vi "libssh2_channel_request_pty_ex.vi"(4 "height_px":i32, 5 "height":i32=24, 6 "width_px":i32, 7 "width":i32=80, 8 "error in (no error)":errorcluster, 9 "modes":string, 10 "term":string, 11 "channel":T1) -> (0 "error out":errorcluster)   [LabVIEW 2017, in "libssh2.lvlib"]
doc: "Request a pseudo-terminal on a channel."
uses:
  libssh2.lvlib
  Channel Refnum.ctl
  Acquire Session.vi
  Release Session.vi
  Not A Channel.vi
  <vilib>/Utility/error.llb/Error Cluster From Error Code.vi
  Global Settings.vi
  Read Channel Refnum.vi
  Read Session Refnum.vi
  <vilib>/Utility/semaphor.llb/Acquire Semaphore.vi
  <vilib>/Utility/semaphor.llb/Release Semaphore.vi
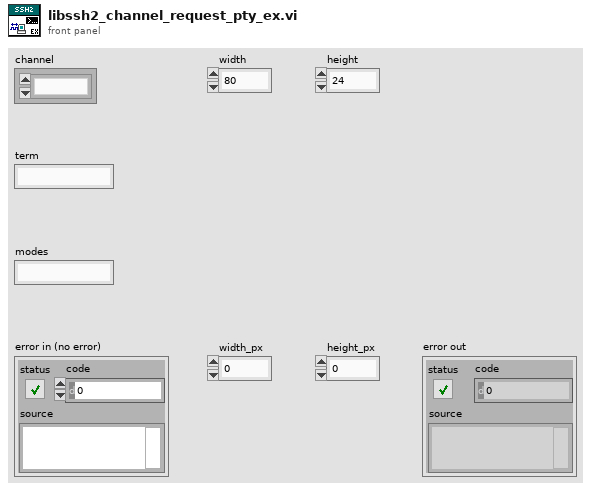
[diagram p1: front panel]
types:
  T1 = typedef "libssh2.lvlib/Channel Refnum.ctl" = refnum<k1>
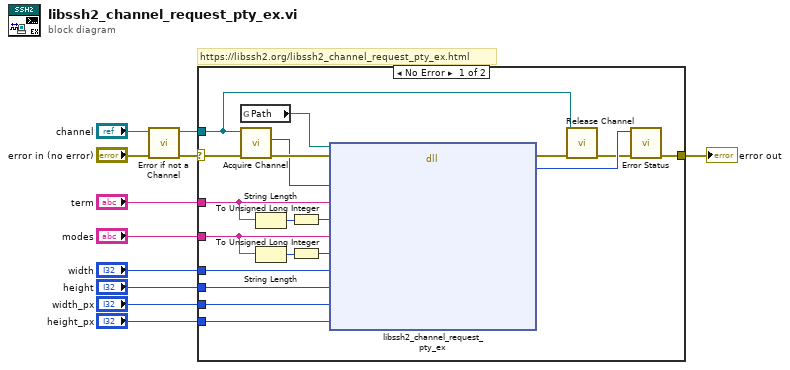
[diagram p0: block diagram]
diagram:
  # "https://libssh2.org/libssh2_channel_request_pty_ex.html"
  n1 = call "Error if not a Channel.vi"("error in (no error)"="error in (no error)", "channel"="channel") -> ("error out"=w9:errorcluster, "channel out"=w7:T1)  [unwired: 8 in]
  n2 = case shown="No Error" w9 {
    selector: w9 -> [w30 w31]
    tunnel: [w29 w31] -> w11
    tunnel: w7 -> [w12 _]
    tunnel: "term" -> [w14 _]
    tunnel: "modes" -> [w18 _]
    tunnel: "width" -> [w23 _]
    tunnel: "height" -> [w22 _]
    tunnel: "width_px" -> [w21 _]
    tunnel: "height_px" -> [w20 _]
    frame No Error {
      n3 = global read "Global Settings.vi" "Path"() -> (w25:path)
      n4 = call "Acquire Channel.vi"("error in (no error)"=w30, "channel"=w12) -> ("error out"=w27:errorcluster, "LIBSSH2_CHANNEL*"=w26:u64)  [unwired: 8 in]
      n5 = String Length(string=w14) -> (length=w16:i32)
      n6 = String Length(string=w18) -> (length=w19:i32)
      n7 = To Unsigned Long Integer(number=w16) -> (unsigned 32bit integer=w15:u32)
      n8 = To Unsigned Long Integer(number=w19) -> (unsigned 32bit integer=w17:u32)
      n9 = dll-call lib="?" fn="libssh2_channel_request_pty_ex"(path in=w25, error in=w27, "channel"=w26, "term"=w14, "term_len"=w15, "modes"=w18, "modes_len"=w17, "width"=w23, "height"=w22, "width_px"=w21, "height_px"=w20) -> (error out=w28:errorcluster, "return value"=w24:i32)  [unwired: 10 in, 1 out]
      n10 = call "Release Channel.vi"("error in (no error)"=w28, "channel"=w12) -> ("error out"=w13:errorcluster)  [unwired: 9 in]
      n11 = call "Error Status.vi"("error in (no error)"=w13, "return value"=w24) -> ("error out"=w29:errorcluster)  [unwired: 8 in, 1 out]
    }
    frame Error {
    }
  }
  "error out" <- w11
